vi "降采样率.vi"() -> ()   [LabVIEW 2023]
uses:
  <vilib>/Analysis/2dsp.llb/Decimate (continuous, DBL).vi
  <vilib>/Analysis/NI_AALPro.lvlib
panel:
  in  "水平指针滑动杆（Horizontal Pointer Slider）":dbl(slide) scale=0.0..2000.0
  out "XY图":T1(graph)
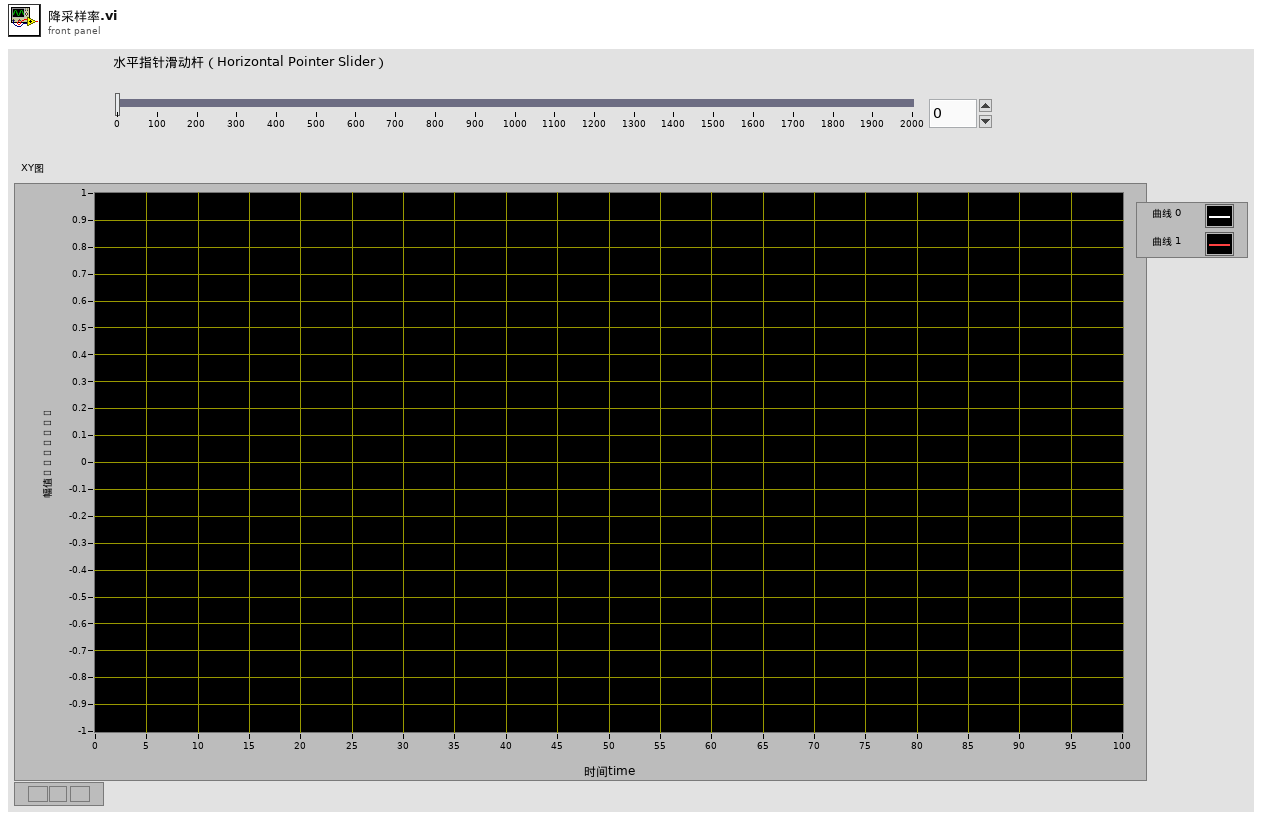
[diagram p1: front panel]
types:
  T1 = cluster{"Decimated Array":dbl[], "Decimated Array":dbl[]}[]
  T2 = cluster{"Decimated Array":dbl[], "Decimated Array":dbl[]}
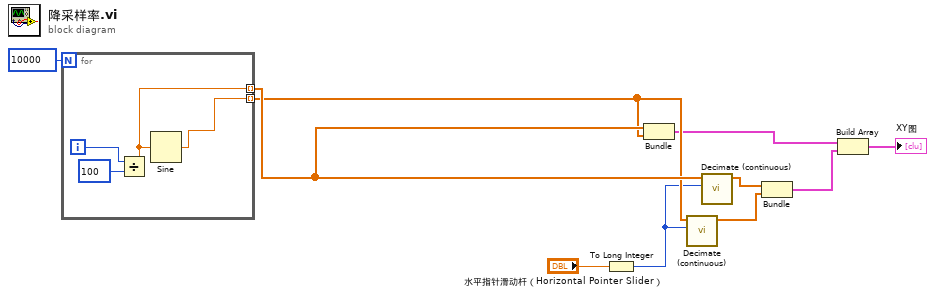
[diagram p0: block diagram]
diagram:
  n1 = for {
    N: 10000 -> [_]
    tunnel: [w12] -> w9 mode=indexing
    tunnel: [w11] -> w8 mode=indexing
    i -> [w14]
    n2 = Divide(x=w14, y=100) -> (x/y=w12:dbl)
    n3 = Sine(x=w12) -> (sin(x)=w11:dbl)
  }
  n4 = To Long Integer(number="水平指针滑动杆（Horizontal Pointer Slider）") -> (32bit integer=w2:i32)
  n5 = Bundle(w9, w8) -> (w5:cluster{dbl[], dbl[]})  [unwired: 1 in]
  n6 = call-poly <vilib>:"Decimate (continuous).vi"("decimating factor"=w2, "X"=w8) -> ("Decimated Array"=w6:dbl[])  [unwired: 8 in, 1 out]
  n7 = call-poly <vilib>:"Decimate (continuous).vi"("decimating factor"=w2, "X"=w9) -> ("Decimated Array"=w7:dbl[])  [unwired: 8 in, 1 out]
  n8 = Bundle("Decimated Array"=w7, "Decimated Array"=w6) -> (w4:T2)  [unwired: 1 in]
  n9 = Build Array(w5, w4) -> (→"XY图":T1)
